vi "VIH UI - String Shortcut Menu Handler.vi"(6 "Project Tree":T2, 7 "mode":enum16{"basic", "format 1", "format 2"}(ring), 8 "Menu tag":string, 9 "menu":refnum<k9>, 10 "Str Refnum":refnum<vi>, 11 "Type":T1) -> ()   [LabVIEW 2014]
doc: "::: VI Helpeks :::\nCopyright (c) 2000-2026 Konstantin Shifershteyn. All rights reserved."
uses:
  VIH Project Tree Typedef - Tree Refnum.ctl
  <vilib>/event_ctls.llb/lveventtype.ctl
  _VIH Support Library.llb/VIH Utility - MENU - Create Menu (String).vi
panel:
  # "VI Helpeks\nCopyright (c) 2012-2026 Konstantin Shifershteyn"
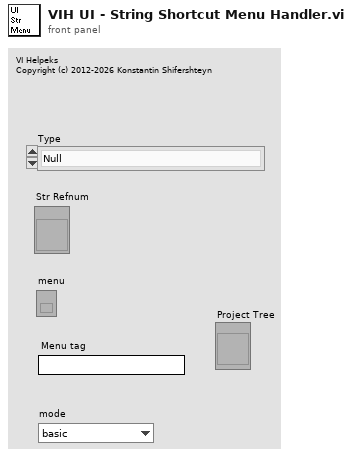
[diagram p1: front panel]
types:
  T1 = typedef "lveventtype.ctl" = enum32{"Null", "Timeout", "Annotation Menu Selection", "Annotation Menu Selection?", "App Instance Close", "App Instance Close?", "Autoscale Range Change", "Bookmark Info Change", "Cell Edit", "Cell Edit?", "Cursor Grab", "Cursor Grab?", "Cursor Menu Selection", "Cursor Menu Selection?", "Cursor Move", "Cursor Release", "Data Change", "Direction Change", "Display State Change", "Drag Ended", "Drag Enter", "Drag Leave", "Drag Over", "Drag Source Update", "Drag Starting", "Drag Starting?", "Drop", "Exec State Change", "Key Down", "Key Down?", "Key Repeat", "Key Repeat?", "Key Up", "Listbox Double Click", "Menu Activation?", "Menu Selection (App)", "Menu Selection? (App)", "Menu Selection (User)", "Mouse Down", "Mouse Down?", "Mouse Enter", "Mouse Leave", "Mouse Move", "Mouse Up", "Mouse Wheel", "NI Security User Change (App)", "Pane Size", "Panel Close", "Panel Close?", "Panel Resize", "Plot Attribute Change", "Scale Range Change", "Shortcut Menu Activation?", "Shortcut Menu Selection (App)", "Shortcut Menu Selection? (App)", "Shortcut Menu Selection (User)", "Tree Double Click", "Tree Drag", "Tree Drag?", "Tree Drop", "Tree Drop?", "Tree Item Close", "Tree Item Close?", "Tree Item Open", "Tree Item Open?", "User Event", "Value Change"}
  T2 = typedef "VIH Project Tree Typedef - Tree Refnum.ctl" = refnum<vi>
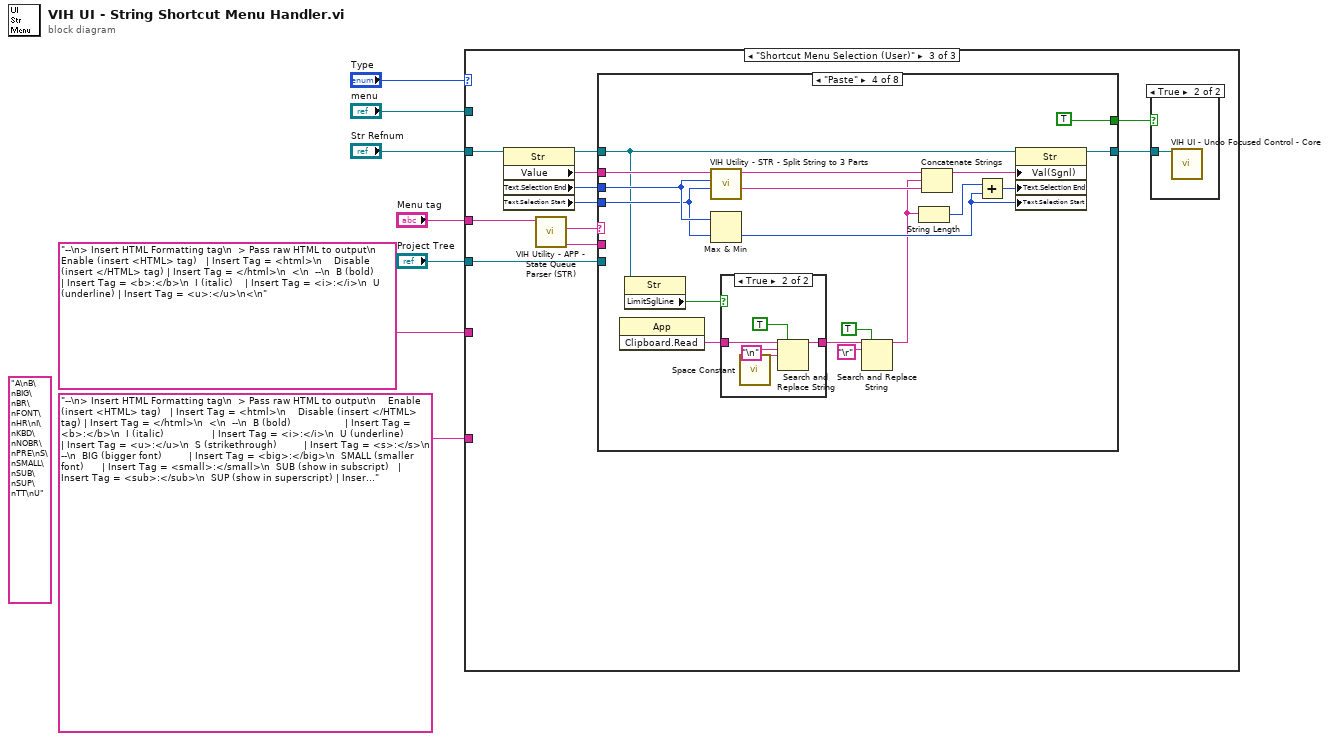
[diagram p0: block diagram]
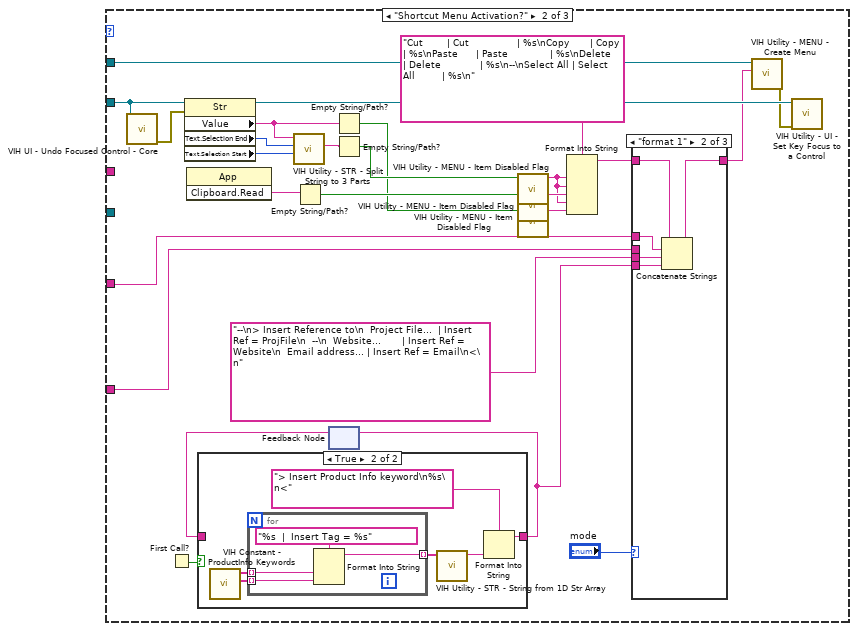
[diagram p3: hidden frame]
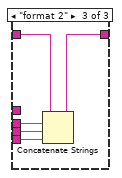
[diagram p6: hidden frame]
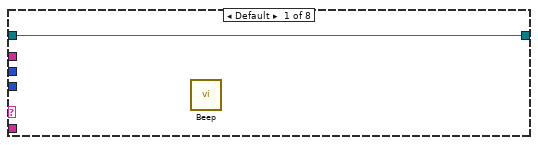
[diagram p8: hidden frame]
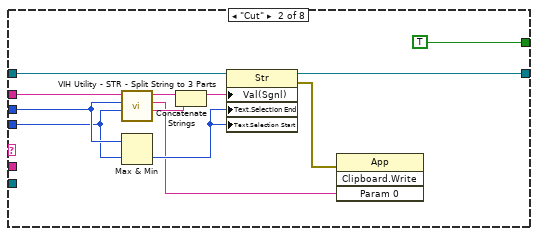
[diagram p9: hidden frame]
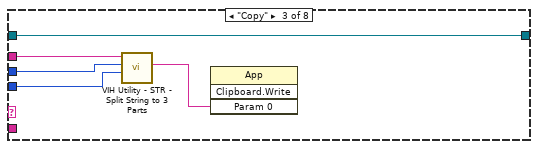
[diagram p10: hidden frame]
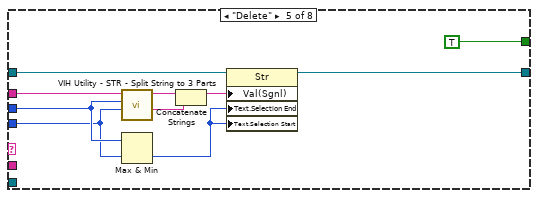
[diagram p12: hidden frame]
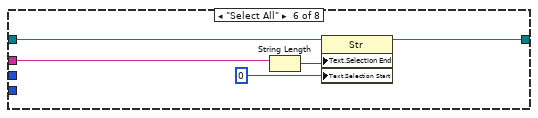
[diagram p13: hidden frame]
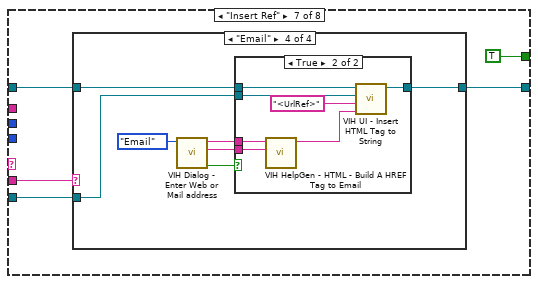
[diagram p14: hidden frame]
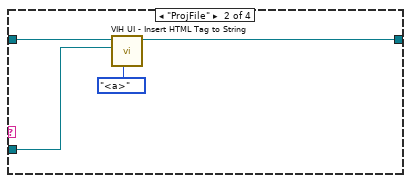
[diagram p16: hidden frame]
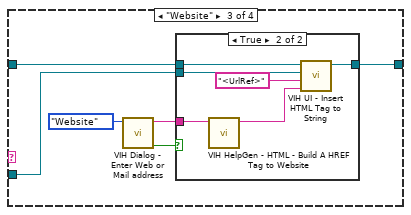
[diagram p17: hidden frame]
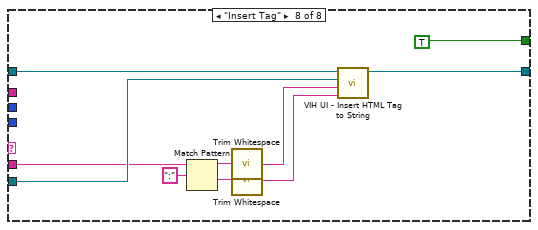
[diagram p20: hidden frame]
diagram:
  (unwired) "A\nB\nBIG\nBR\nFONT\nHR\nI\nKBD\nNOBR\nPRE\nS\nSMALL\nSUB\nSUP\nTT\nU" ("String in")
  n1 = case shown="\"Shortcut Menu Selection (User)\"" "Type" {
    tunnel: "Str Refnum" -> [_ w9 w62]
    tunnel: "menu" -> [_ w20 _]
    tunnel: "Project Tree" -> [_ _ w64]
    tunnel: "Menu tag" -> [_ _ w63]
    tunnel: "--\n> Insert HTML Formatting tag\n  > Pass raw HTML to output\n    Enable (insert <HTML> tag)   | Insert Tag = <html>\n    Disable (insert </HTML> tag) | Insert Tag = </html>\n  <\n  --\n  B (bold)      | Insert Tag = <b>:</b>\n  I (italic)    | Insert Tag = <i>:</i>\n  U (underline) | Insert Tag = <u>:</u>\n<\n" -> [_ w13 _]
    tunnel: "--\n> Insert HTML Formatting tag\n  > Pass raw HTML to output\n    Enable (insert <HTML> tag)   | Insert Tag = <html>\n    Disable (insert </HTML> tag) | Insert Tag = </html>\n  <\n  --\n  B (bold)                  | Insert Tag = <b>:</b>\n  I (italic)                | Insert Tag = <i>:</i>\n  U (underline)             | Insert Tag = <u>:</u>\n  S (strikethrough)         | Insert Tag = <s>:</s>\n  --\n  BIG (bigger font)         | Insert Tag = <big>:</big>\n  SMALL (smaller font)      | Insert Tag = <small>:</small>\n  SUB (show in subscript)   | Insert Tag = <sub>:</sub>\n  SUP (show in superscript) | Insert Tag = <sup>:</sup>\n  --\n  BR (line brake)           | Insert Tag = <br>\n  HR (horizontal rule)      | Insert Tag = <hr>\n  NOBR (disable line break) | Insert Tag = <nobr>:</nobr>\n  --\n  KBD (keyboard input)      | Insert Tag = <kbd>:</kbd>\n  PRE (fixed-width & preserve)    | Insert Tag = <pre>:</pre>\n  TT (teletype text)        | Insert Tag = <tt>:</tt>\n  --\n  FONT (font attributes)    | Insert Tag = <font>:</font>\n<\n" ("String in") -> [_ w12 _]
    frame "Null", Default {
    }
    frame "Shortcut Menu Activation?" {
      n2 = call "VIH UI - Undo Focused Control - Core.vi"("Ctl Refnum"=w9) -> ("no error out"=w8:errorcluster)  [unwired: 8 in, 2 out]
      n3 = First Call?() -> (First Call?: T/F=w15:bool)
      n4 = property on="Property Node" class="Str"(reference=w9, error in=w8) -> (reference out=w30:refnum<vi>, "Value"=w29:string, "Text.Selection End"=w32:u32, "Text.Selection Start"=w31:u32)  [unwired: 1 out]
      n5 = invoke class="App" method="Clipboard.Read"() -> ("Read Clipbrd"=w24:string)  [unwired: 3 in, 2 out]
      n6 = call "VIH Utility - STR - Split String to 3 Parts.vi"("Position 2"=w31, "Position 1"=w32, "String"=w29) -> ("Middle"=w28:string)  [unwired: 6 in, 2 out]
      n7 = Empty String/Path?(string/path=w24) -> (empty?=w25:bool)
      n8 = feedback #1() -> (w14:string)  [unwired: 1 in]
      n9 = case shown="True" w15 {
        tunnel: [w34 w35] -> w10
        tunnel: w14 -> [w34 _]
        frame False {
        }
        frame True {
          n10 = call "VIH Constant - ProductInfo Keywords.vi"() -> ("ProductInfo keywords"=w38:string[], "Keyword description"=w39:string[])  [unwired: 10 in]
          n11 = for {
            tunnel: w39 -> [w43] mode=indexing
            tunnel: w38 -> [w42] mode=indexing
            tunnel: [w41] -> w37 mode=indexing
            n12 = Format Into String(format string="%s  |  Insert Tag = %s", w43, w42) -> (resulting string=w41:string)  [unwired: 2 in, 1 out]
          }
          n13 = call "VIH Utility - STR - String from 1D Str Array.vi"("Array in"=w37) -> ("String out"=w36:string)  [unwired: 6 in]
          n14 = Format Into String(format string="> Insert Product Info keyword\n%s\n<", w36) -> (resulting string=w35:string)  [unwired: 2 in, 1 out]
        }
      }
      n15 = feedback-in #1(w10) -> ()
      n16 = Empty String/Path?(string/path=w29) -> (empty?=w22:bool)
      n17 = Empty String/Path?(string/path=w28) -> (empty?=w27:bool)
      n18 = call "VIH Utility - MENU - Item Disabled Flag.vi"("Disable?"=w27) -> ("Disable flag"=w19:string)  [unwired: 10 in]
      n19 = call "VIH Utility - MENU - Item Disabled Flag.vi"("Disable?"=w25) -> ("Disable flag"=w26:string)  [unwired: 10 in]
      n20 = call "VIH Utility - MENU - Item Disabled Flag.vi"("Disable?"=w22) -> ("Disable flag"=w23:string)  [unwired: 10 in]
      n21 = Format Into String(format string="Cut        | Cut                | %s\nCopy       | Copy               | %s\nPaste      | Paste              | %s\nDelete     | Delete             | %s\n--\nSelect All | Select All         | %s\n", w19, w19, w26, w19, w23) -> (resulting string=w18:string)  [unwired: 2 in, 1 out]
      n22 = case shown="\"format 1\"" "mode" {
        tunnel: w18 -> [w45 w50 w55]
        tunnel: [w45 w49 w54] -> w17
        tunnel: w13 -> [_ w48 _]
        tunnel: w12 -> [_ _ w53]
        tunnel: "--\n> Insert Reference to\n  Project File...  | Insert Ref = ProjFile\n  --\n  Website...       | Insert Ref = Website\n  Email address... | Insert Ref = Email\n<\n" -> [_ w47 w52]
        tunnel: w10 -> [_ w46 w51]
        frame "basic" {
        }
        frame "format 1" {
          n23 = Concatenate Strings(w50, w48, w47, w46) -> (w49:string)
        }
        frame "format 2" {
          n24 = Concatenate Strings(w55, w53, w52, w51) -> (w54:string)
        }
      }
      n25 = call-poly "VIH Utility - MENU - Create Menu.vi"("Menu Description"=w17, "menu"=w20) -> ("error out"=w21:errorcluster)  [unwired: 8 in, 1 out]
      n26 = call "VIH Utility - UI - Set Key Focus to a Control.vi"("error in"=w21, "Ctl Refnum"=w30) -> ()  [unwired: 8 in, 2 out]
    }
    frame "Shortcut Menu Selection (User)" {
      n27 = property on="Property Node" class="Str"(reference=w62) -> (reference out=w61:refnum<vi>, "Value"=w60:string, "Text.Selection End"=w59:u32, "Text.Selection Start"=w58:u32)  [unwired: 1 in, 1 out]
      n28 = call "VIH Utility - APP - State Queue Parser (STR).vi"("input queue"=w63) -> ("state parameters"=w66:string, "state"=w65:string)  [unwired: 5 in, 2 out]
      n29 = case shown="\"Paste\"" w65 {
        tunnel: w61 -> [w68 w79 w81 w94 w118 w124 w126 w165]
        tunnel: w64 -> [_ _ _ _ _ _ w129 w172]
        tunnel: w66 -> [_ _ _ _ _ _ w128 w171]
        tunnel: w60 -> [_ w80 w85 w103 w119 w122 _ _]
        tunnel: w59 -> [_ w78 w84 w102 w117 _ _ _]
        tunnel: w58 -> [_ w77 w83 w101 w116 _ _ _]
        tunnel: [w68 w70 w81 w87 w111 w120 w125 w163] -> w57
        tunnel: [_ TRUE _ TRUE TRUE _ TRUE TRUE] -> w56
        frame Default {
          n30 = call <vilib>:"Beep.vi"() -> ()  [unwired: 12 in]
        }
        frame "Cut" {
          n31 = call "VIH Utility - STR - Split String to 3 Parts.vi"("Position 2"=w77, "Position 1"=w78, "String"=w80) -> ("After"=w74:string, "Middle"=w72:string, "Before"=w75:string)  [unwired: 6 in]
          n32 = Max & Min(x=w78, y=w77) -> (min(x,y)=w76:u32)  [unwired: 1 out]
          n33 = Concatenate Strings(w75, w74) -> (w73:string)
          n34 = property on="Property Node" class="Str"(reference=w79, "Val(Sgnl)"=w73, "Text.Selection End"=w76, "Text.Selection Start"=w76) -> (reference out=w70:refnum<vi>, error out=w71:errorcluster)  [unwired: 1 in]
          n35 = invoke class="App" method="Clipboard.Write"(error in=w71, "Param 0"=w72) -> ()  [unwired: 2 in, 4 out]
        }
        frame "Copy" {
          n36 = call "VIH Utility - STR - Split String to 3 Parts.vi"("Position 2"=w83, "Position 1"=w84, "String"=w85) -> ("Middle"=w82:string)  [unwired: 6 in, 2 out]
          n37 = invoke class="App" method="Clipboard.Write"("Param 0"=w82) -> ()  [unwired: 3 in, 4 out]
        }
        frame "Paste" {
          n38 = invoke class="App" method="Clipboard.Read"() -> ("Read Clipbrd"=w92:string)  [unwired: 3 in, 2 out]
          n39 = property class="Str"(reference=w94) -> ("LimitSglLine"=w93:bool)  [unwired: 1 in, 2 out]
          n40 = call "VIH Utility - STR - Split String to 3 Parts.vi"("Position 2"=w101, "Position 1"=w102, "String"=w103) -> ("After"=w99:string, "Before"=w100:string)  [unwired: 6 in, 1 out]
          n41 = Max & Min(x=w102, y=w101) -> (min(x,y)=w97:u32)  [unwired: 1 out]
          n42 = case shown="True" w93 {
            tunnel: w92 -> [w104 w109]
            tunnel: [w104 w105] -> w91
            frame False {
            }
            frame True {
              n43 = call <vilib>:"Space Constant.vi"() -> ("String"=w106:string)
              n44 = Search and Replace String(replace all?=TRUE, input string=w109, search string="\n", replace string=w106) -> (result string=w105:string)  [unwired: 4 in, 3 out]
            }
          }
          n45 = Search and Replace String(replace all?=TRUE, input string=w91, search string="\r") -> (result string=w88:string)  [unwired: 5 in, 3 out]
          n46 = String Length(string=w88) -> (length=w95:i32)
          n47 = Concatenate Strings(w100, w88, w99) -> (w98:string)
          n48 = Add(x=w95, y=w97) -> (x+y=w96:u32)
          n49 = property on="Property Node" class="Str"(reference=w94, "Val(Sgnl)"=w98, "Text.Selection End"=w96, "Text.Selection Start"=w97) -> (reference out=w87:refnum<vi>)  [unwired: 1 in, 1 out]
        }
        frame "Delete" {
          n50 = call "VIH Utility - STR - Split String to 3 Parts.vi"("Position 2"=w116, "Position 1"=w117, "String"=w119) -> ("After"=w113:string, "Before"=w114:string)  [unwired: 6 in, 1 out]
          n51 = Max & Min(x=w117, y=w116) -> (min(x,y)=w115:u32)  [unwired: 1 out]
          n52 = Concatenate Strings(w114, w113) -> (w112:string)
          n53 = property on="Property Node" class="Str"(reference=w118, "Val(Sgnl)"=w112, "Text.Selection End"=w115, "Text.Selection Start"=w115) -> (reference out=w111:refnum<vi>)  [unwired: 1 in, 1 out]
        }
        frame "Select All" {
          n54 = String Length(string=w122) -> (length=w121:i32)
          n55 = property on="Property Node" class="Str"(reference=w124, "Text.Selection End"=w121, "Text.Selection Start"=u32 0 ("Text.Selection:Start")) -> (reference out=w120:refnum<vi>)  [unwired: 1 in, 1 out]
        }
        frame "Insert Ref" {
          n56 = case shown="\"Email\"" w128 {
            tunnel: w126 -> [w130 w134 w140 w154]
            tunnel: w129 -> [_ w133 w139 w153]
            tunnel: [w130 w131 w135 w148] -> w125
            frame Default {
            }
            frame "ProjFile" {
              n57 = call "VIH UI - Insert HTML Tag to String.vi"("cmd"=enum32{"nop", "<a>", "<b>", "<i>", "<u>"}."<a>", "Project Tree"=w133, "Str Refnum"=w134) -> ("dup Str Refnum"=w131:refnum<vi>)  [unwired: 8 in]
            }
            frame "Website" {
              n58 = call "VIH Dialog - Enter Web or Mail address.vi"("Type"=enum16{"Website", "Email"}."Website") -> ("OK out"=w136:bool, "Address out"=w137:string)  [unwired: 8 in, 1 out]
              n59 = case shown="True" w136 {
                tunnel: w140 -> [w141 w147]
                tunnel: w139 -> [_ w146]
                tunnel: w137 -> [_ w145]
                tunnel: [w141 w142] -> w135
                frame False {
                }
                frame True {
                  n60 = call "VIH HelpGen - HTML - Build A HREF Tag to Website.vi"("URL"=w145) -> ("HTML tag"=w143:string)  [unwired: 10 in]
                  n61 = call "VIH UI - Insert HTML Tag to String.vi"("tag 2"=w143, "tag 1"="<UrlRef>", "Project Tree"=w146, "Str Refnum"=w147) -> ("dup Str Refnum"=w142:refnum<vi>)  [unwired: 7 in]
                }
              }
            }
            frame "Email" {
              n62 = call "VIH Dialog - Enter Web or Mail address.vi"("Type"=enum16{"Website", "Email"}."Email") -> ("OK out"=w150:bool, "Subject out"=w151:string, "Address out"=w152:string)  [unwired: 8 in]
              n63 = case shown="True" w150 {
                tunnel: w154 -> [w155 w162]
                tunnel: w153 -> [_ w161]
                tunnel: w152 -> [_ w159]
                tunnel: w151 -> [_ w157]
                tunnel: [w155 w156] -> w148
                frame False {
                }
                frame True {
                  n64 = call "VIH HelpGen - HTML - Build A HREF Tag to Email.vi"("Subject"=w157, "Email address"=w159) -> ("HTML tag"=w158:string)  [unwired: 9 in]
                  n65 = call "VIH UI - Insert HTML Tag to String.vi"("tag 2"=w158, "tag 1"="<UrlRef>", "Project Tree"=w161, "Str Refnum"=w162) -> ("dup Str Refnum"=w156:refnum<vi>)  [unwired: 7 in]
                }
              }
            }
          }
        }
        frame "Insert Tag" {
          n66 = Match Pattern(string=w171, regular expression=":") -> (before substring=w169:string, after substring=w168:string)  [unwired: 1 in, 2 out]
          n67 = call <vilib>:"Trim Whitespace.vi"("string"=w169) -> ("trimmed string"=w167:string)  [unwired: 1 in]
          n68 = call <vilib>:"Trim Whitespace.vi"("string"=w168) -> ("trimmed string"=w166:string)  [unwired: 1 in]
          n69 = call "VIH UI - Insert HTML Tag to String.vi"("tag 2"=w166, "tag 1"=w167, "Project Tree"=w172, "Str Refnum"=w165) -> ("dup Str Refnum"=w163:refnum<vi>)  [unwired: 7 in]
        }
      }
      n70 = case shown="True" w56 {
        tunnel: w57 -> [_ w67]
        frame False {
        }
        frame True {
          n71 = call "VIH UI - Undo Focused Control - Core.vi"("Ctl Refnum"=w67) -> ()  [unwired: 8 in, 3 out]
        }
      }
    }
  }
